vi "JSON_coords_translate (SubVI).vi"(5 "Altitude, m":dbl, 7 "Speed, mph":dbl, 8 "error in":errorcluster, 11 "Coordinates string (in)":string) -> (0 "error out":errorcluster, 1 "Coordinates string (out)":string, 3 "waypoints file path":path)   [LabVIEW 2025]
panel:
  out "Lon substring array (debug)":string[](array[string])
  out "Lat substring array (debug)":string[](array[string])
  # "JSON to waypoints coordinates file translation SubVI"
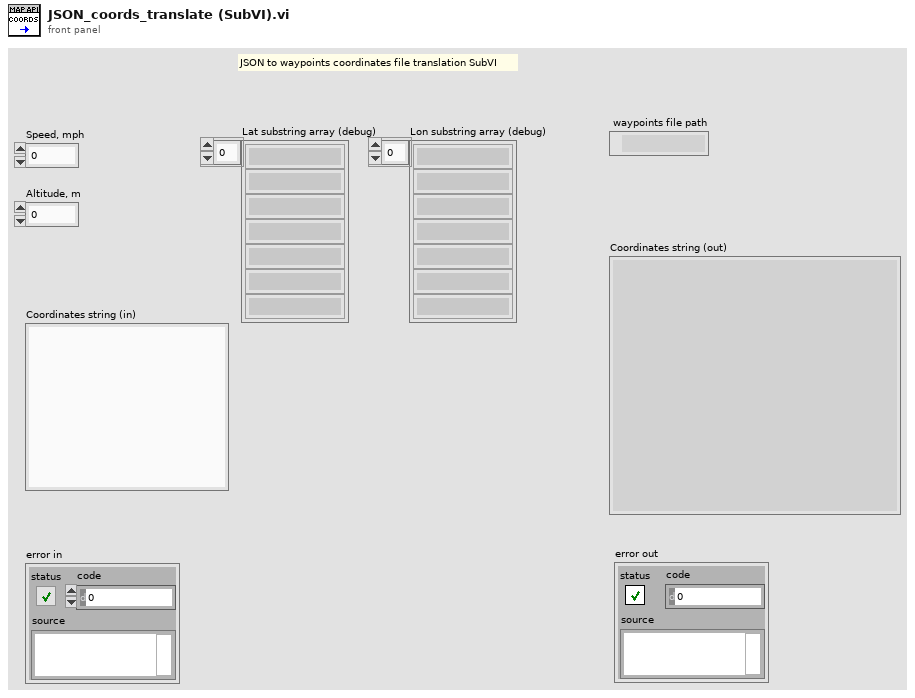
[diagram p1: front panel]
types:
  T1 = enum16{"open", "replace", "create", "open or create", "replace or create", "replace or create with confirmation"}
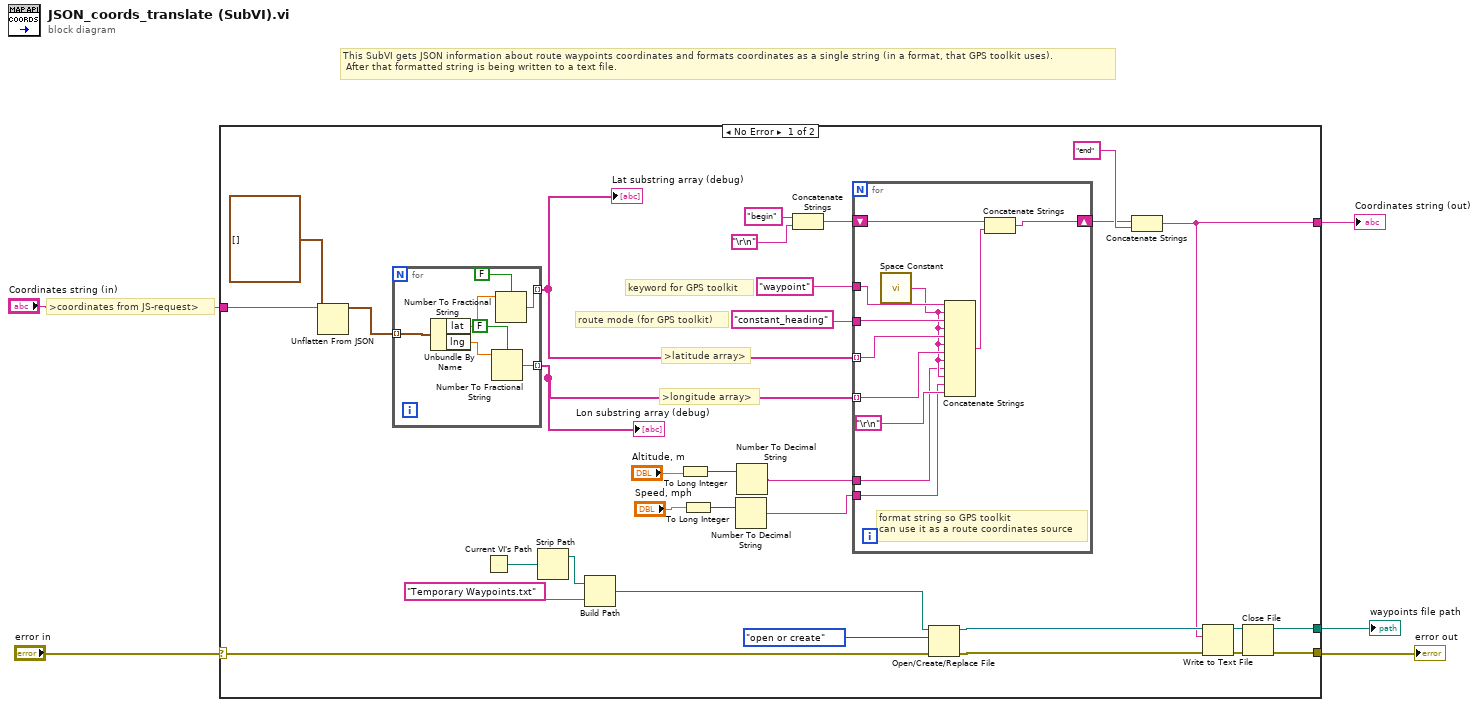
[diagram p0: block diagram]
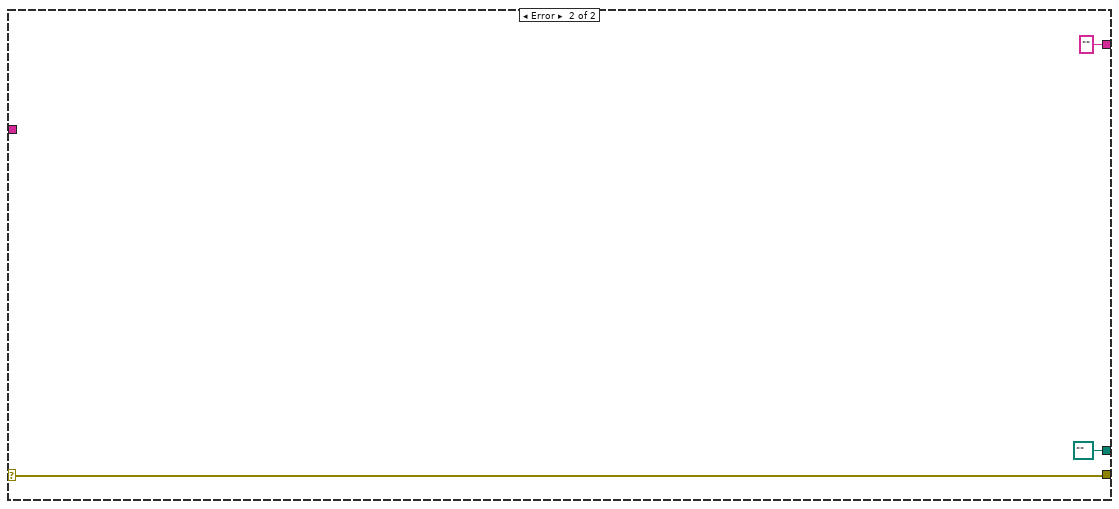
[diagram p2: hidden frame]
diagram:
  # ">coordinates from JS-request>"
  # "This SubVI gets JSON information about route waypoints coordinates and formats coordinates as a single string (in a format, that GPS toolkit uses).\n After that formatted string is being written to a text file."
  n1 = case shown="No Error" "error in" {
    selector: "error in" -> [w20 w57]
    tunnel: [w32 w57] -> w5
    tunnel: "Coordinates string (in)" -> [w19 _]
    tunnel: [w14 ""] -> w2
    tunnel: [w13 path "" ("path")] -> w1
    frame No Error {
      # "keyword for GPS toolkit"
      # "route mode (for GPS toolkit)"
      # ">latitude array>"
      # ">longitude array>"
      n2 = Unflatten From JSON(JSON string=w19, type and defaults=cluster{"lat":ext, "lng":ext}[] []) -> (value=w17:cluster{"lat":ext, "lng":ext}[])  [unwired: 5 in, 1 out]
      n3 = for {
        tunnel: w17 -> [w43] mode=indexing
        tunnel: [w40] -> w16 mode=indexing
        tunnel: [w39] -> w15 mode=indexing
        n4 = Unbundle By Name(w43) -> ("lat"=w42:ext, "lng"=w41:ext)
        n5 = Number To Fractional String(use system decimal point (T)=FALSE, number=w41) -> (F-format string=w39:string)  [unwired: 2 in]
        n6 = Number To Fractional String(use system decimal point (T)=FALSE, number=w42) -> (F-format string=w40:string)  [unwired: 2 in]
      }
      "Lat substring array (debug)" <- w16
      "Lon substring array (debug)" <- w15
      n7 = Current VI's Path() -> (path=w22:path)
      n8 = Strip Path(path=w22) -> (stripped path=w31:path)  [unwired: 1 out]
      n9 = Build Path(base path=w31, name or relative path="Temporary Waypoints.txt") -> (appended path=w12:path)
      n10 = To Long Integer(number="Altitude, m") -> (32bit integer=w6:i32)
      n11 = To Long Integer(number="Speed, mph") -> (32bit integer=w8:i32)
      n12 = Number To Decimal String(number=w8) -> (decimal integer string=w10:string)  [unwired: 1 in]
      n13 = Number To Decimal String(number=w6) -> (decimal integer string=w11:string)  [unwired: 1 in]
      n14 = Concatenate Strings("begin", "\r\n") -> (w25:string)
      n15 = for {
        tunnel: w15 -> [w51] mode=indexing
        tunnel: w16 -> [w52] mode=indexing
        tunnel: "waypoint" -> [w54]
        tunnel: "constant_heading" -> [w53]
        tunnel: w11 -> [w44]
        tunnel: w10 -> [w45]
        shift-right: [w46] -> w23
        shift-left: w25 -> [w48]
        # "format string so GPS toolkit \ncan use it as a route coordinates source"
        n16 = call <vilib>:"Space Constant.vi"() -> ("String"=w50:string)
        n17 = Concatenate Strings(w54, w50, w53, w50, w52, w50, w51, w50, w44, w50, w45, "\r\n") -> (w47:string)
        n18 = Concatenate Strings(w48, w47) -> (w46:string)
      }
      n19 = Open/Create/Replace File(file path (use dialog)=w12, error in=w20, operation (0:open)=T1."open or create") -> (refnum out=w36:refnum<file>, error out=w34:errorcluster)  [unwired: 4 out]
      n20 = Concatenate Strings(w23, "end") -> (w14:string)
      n21 = Write to Text File(file (use dialog)=w36, text=w14, error in=w34) -> (refnum out=w35:refnum<file>, error out=w33:errorcluster)  [unwired: 2 out]
      n22 = Close File(refnum=w35, error in=w33) -> (path=w13:path, error out=w32:errorcluster)
    }
    frame Error {
    }
  }
  "error out" <- w5
  "Coordinates string (out)" <- w2
  "waypoints file path" <- w1
